vi "Get SLSC Module Resource from Chassis IP.vi"(5 "Password":string, 7 "Username":string, 8 "error in (no error)":errorcluster, 10 "Slot Number":i32, 11 "Chassis Name or IP":string) -> (0 "error out":errorcluster, 3 "SLSC Device":refnum<k21>)   [LabVIEW 2020, in "VeriStand SLSC Scripting.lvlib"]
uses:
  VeriStand SLSC Scripting.lvlib
  <vilib>/nisyscfg/Close (System).vi
  <vilib>/SLSC/Initialize Session with Devices.vi
  <vilib>/SLSC/Initialize Session without Resources.vi
  <vilib>/SLSC/Close Session.vi
  <vilib>/nisyscfg/nisyscfg.lvlib
  <resource>/objmgr/nisysapi.rc
  <vilib>/SLSC/SLSC.lvlib
  <resource>/objmgr/slsc.rc
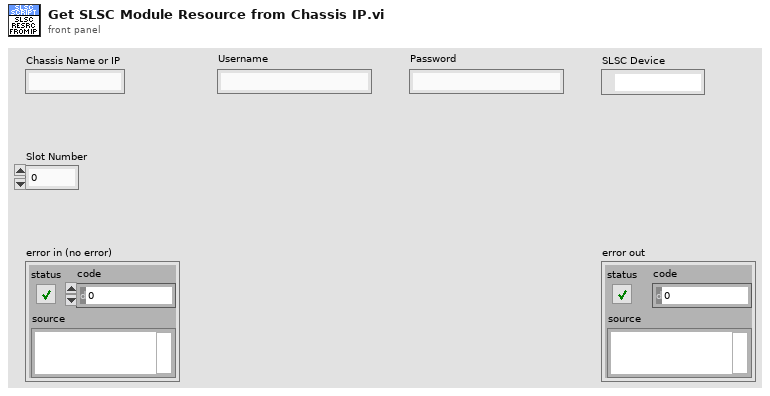
[diagram p1: front panel]
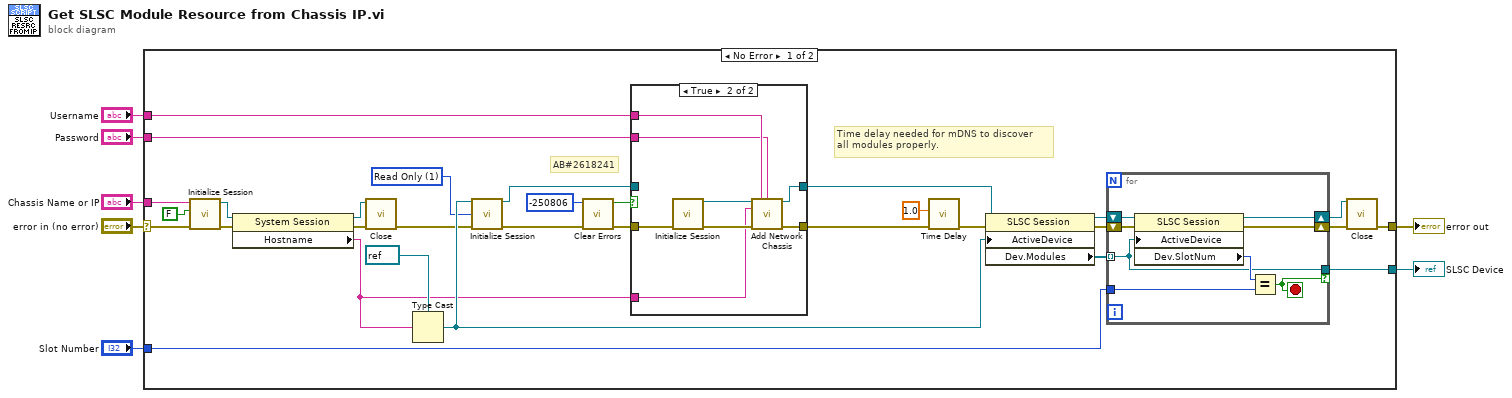
[diagram p0: block diagram]
diagram:
  n1 = case shown="No Error" "error in (no error)" {
    selector: "error in (no error)" -> [w36 w57]
    tunnel: "Chassis Name or IP" -> [w38 _]
    tunnel: [w35 w57] -> w5
    tunnel: [w32 _] -> w4
    tunnel: "Slot Number" -> [w31 _]
    tunnel: "Username" -> [w9 _]
    tunnel: "Password" -> [w8 _]
    frame No Error {
      w25 = 1 items=["None"=0, "Read Only"=1, "Read/Write"=3] ("reservation access (Read/Write)")
      # "AB#2618241"
      # "Time delay needed for mDNS to discover\nall modules properly."
      n2 = call <vilib>:"Initialize Session.vi"("error in (no error)"=w36, "Force Property Refresh (T)"=FALSE, "Target (localhost)"=w38) -> ("error out"=w21:errorcluster, "Session out"=w20:refnum<k21>)  [unwired: 7 in]
      n3 = property class="System Session"(reference=w20, error in=w21) -> (reference out=w24:refnum<k21>, error out=w22:errorcluster, "Hostname"=w11:string)
      n4 = call-poly <vilib>:"Close.vi"("error in (no error)"=w22, "Session in"=w24) -> ("error out"=w26:errorcluster)  [unwired: 9 in]
      n5 = Type Cast(type=refnum<k21> refnum ("devices"), x=w11) -> (*(type *) &x=w28:refnum<k21>)
      n6 = call-poly <vilib>:"Initialize Session.vi"("devices"=w28, "reservation access (Read/Write)"=w25, "error in (no error)"=w26) -> ("session out"=w12:refnum<k21>, "error out"=w17:errorcluster)  [unwired: 11 in]
      n7 = call <vilib>:"Clear Errors.vi"("error in (no error)"=w17, "specific error code to clear (0: all)"=-250806) -> ("error out"=w14:errorcluster, "specific error cleared?"=w15:bool)  [unwired: 4 in]
      n8 = case shown="True" w15 {
        tunnel: w14 -> [w40 w48]
        tunnel: [w40 w47] -> w13
        tunnel: w12 -> [w39 _]
        tunnel: w11 -> [_ w44]
        tunnel: [w39 w43] -> w10
        tunnel: w9 -> [_ w42]
        tunnel: w8 -> [_ w41]
        frame False {
        }
        frame True {
          n9 = call-poly <vilib>:"Initialize Session.vi"("error in (no error)"=w48) -> ("session out"=w45:refnum<k21>, "error out"=w46:errorcluster)  [unwired: 13 in]
          n10 = call <vilib>:"Add Network Chassis.vi"("session in"=w45, "username"=w42, "password"=w41, "chassis IP address/hostname"=w44, "error in (no error)"=w46) -> ("session out"=w43:refnum<k21>, "error out"=w47:errorcluster)  [unwired: 8 in, 1 out]
        }
      }
      n11 = call "Time Delay"("error in (no error)"=w13, "Delay Time (s)"=1.0) -> ("error out"=w18:errorcluster)  [unwired: 9 in]
      n12 = property class="SLSC Session"(reference=w10, error in=w18, "ActiveDevice"=w28) -> (reference out=w29:refnum<k21>, error out=w30:errorcluster, "Dev.Modules"=w37:refnum<k21>[])
      n13 = for {
        tunnel: w37 -> [w49] mode=indexing
        shift-right: [w54] -> w34
        shift-left: w30 -> [w55]
        shift-right: [w53] -> w33
        shift-left: w29 -> [w56]
        tunnel: w31 -> [w51]
        tunnel: [w49] -> w32 if=w50
        stop <- w50 stop-if-true
        n14 = property class="SLSC Session"(reference=w56, error in=w55, "ActiveDevice"=w49) -> (reference out=w53:refnum<k21>, error out=w54:errorcluster, "Dev.SlotNum"=w52:u32)
        n15 = Equal?(x=w52, y=w51) -> (x = y?=w50:bool)
      }
      n16 = call-poly <vilib>:"Close.vi"("session in"=w33, "error in (no error)"=w34) -> ("error out"=w35:errorcluster)  [unwired: 13 in]
    }
    frame Error {
    }
  }
  "error out" <- w5
  "SLSC Device" <- w4
